vi "OverlayArrow.vi"(6 "Color":u32(colorbox)=16711680, 7 "GroupName":string, 8 "error in":errorcluster, 9 "Arrows":T1={"StartPoint"=TRUE, "StartArrowSize"=9.0, "EndPoint"=TRUE, "EndArrowSize"=9.0}, 10 "Line":T2, 11 "Image Reference In":T4) -> (0 "error out":errorcluster, 3 "Image Reference Out":T4)   [LabVIEW 2020, in "OpenLvVision_Overlays.lvlib"]
doc: "Overlays an Arrow into an image."
uses:
  OpenLvVision_Overlays.lvlib
  <vilib>/OpenLvVision/OpenLvVision_Image/Management/TypeDef/OLV Image.ctl
  TypeDefs/Line.ctl
  TypeDefs/PointI32.ctl
  TypeDefs/Arrows.ctl
  TypeDefs/DrawingMode.ctl
  <vilib>/OpenLvVision/OpenLvVision_Image/Management/OLV Management.lvlib
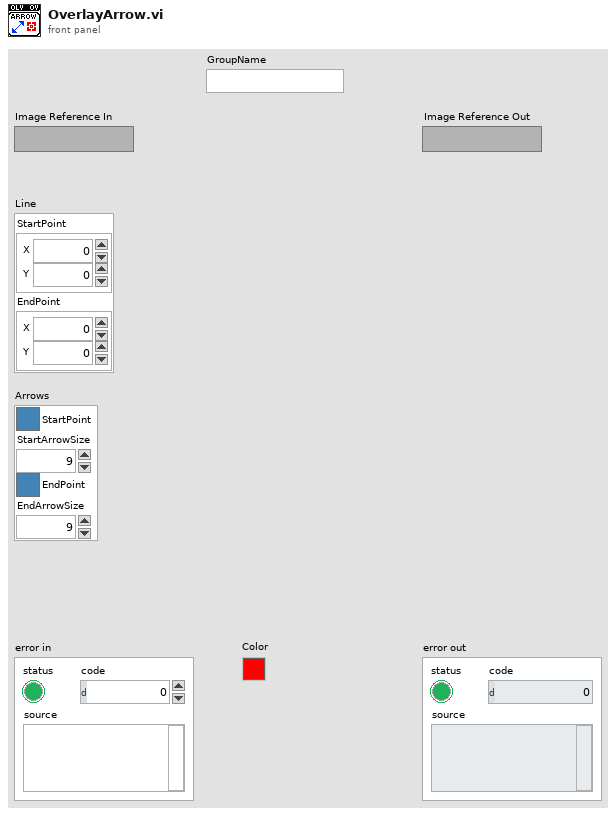
[diagram p1: front panel]
types:
  T1 = typedef "OpenLvVision_Overlays.lvlib/Arrows.ctl" = cluster{"StartPoint":bool, "StartArrowSize":dbl, "EndPoint":bool, "EndArrowSize":dbl}
  T2 = typedef "OpenLvVision_Overlays.lvlib/Line.ctl" = cluster{"StartPoint":T3, "EndPoint":T3}
  T3 = typedef "OpenLvVision_Overlays.lvlib/PointI32.ctl" = cluster{"X":i32, "Y":i32}
  T4 = typedef "OLV OpenLvVision_Image.lvlib/OLV Management.lvlib/OLV Image.ctl" = refnum<image>
  T5 = typedef "OpenLvVision_Overlays.lvlib/DrawingMode.ctl" = enum16{"Frame", "Fill"}
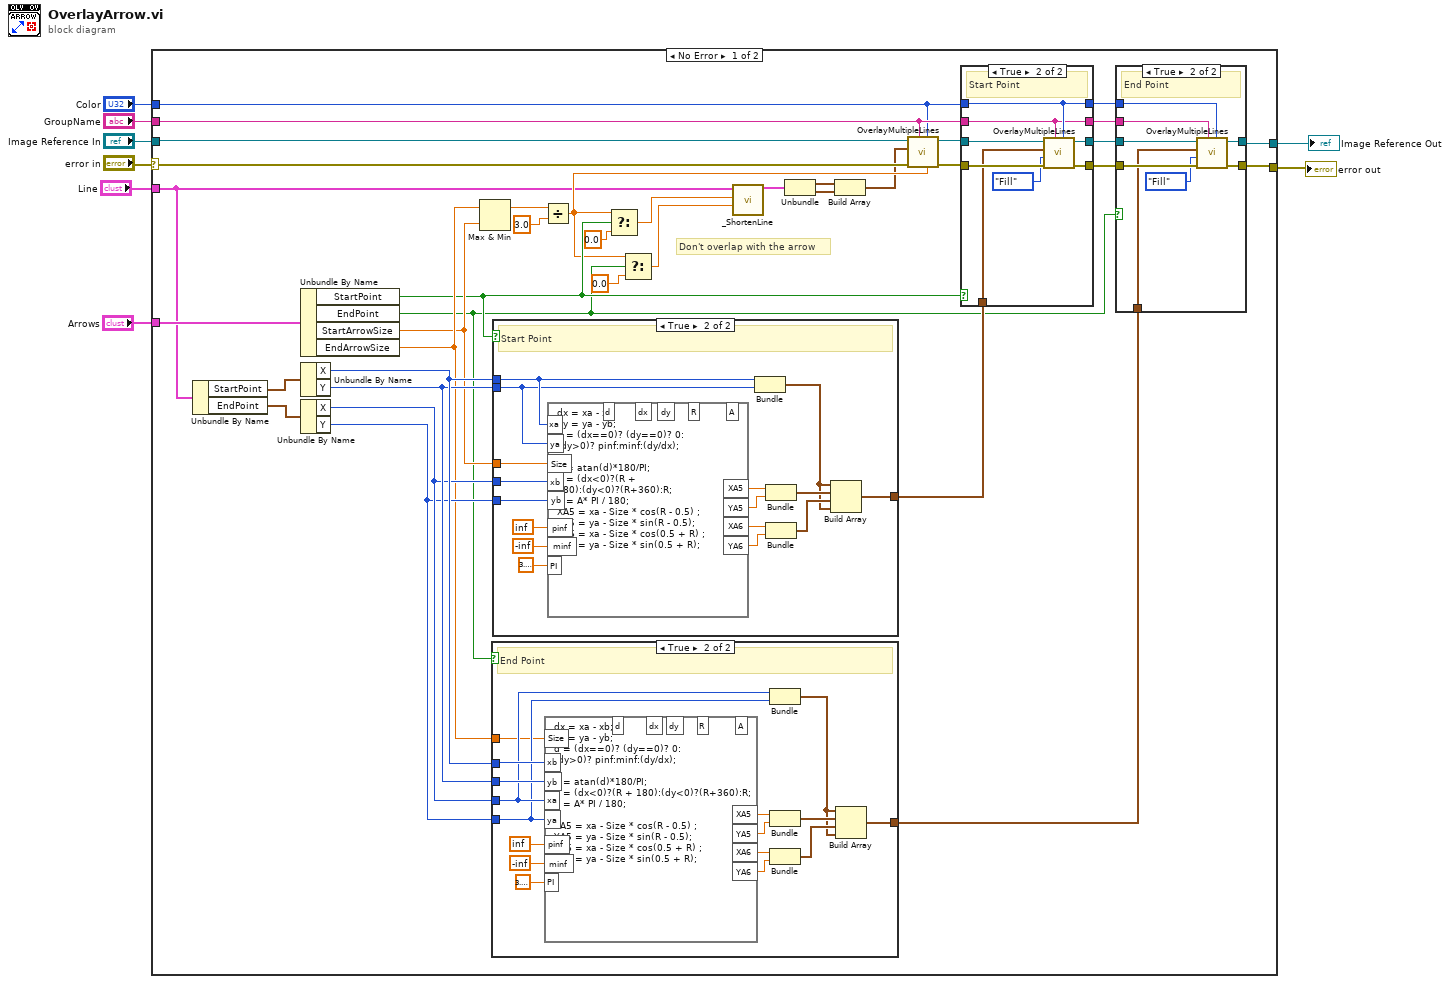
[diagram p0: block diagram]
diagram:
  n1 = case shown="No Error" "error in" {
    selector: "error in" -> [w32 w100]
    tunnel: [w36 w100] -> w7
    tunnel: "Image Reference In" -> [w31 w101]
    tunnel: [w35 w101] -> w6
    tunnel: "Arrows" -> [w45 _]
    tunnel: "Color" -> [w27 _]
    tunnel: "GroupName" -> [w28 _]
    tunnel: "Line" -> [w11 _]
    frame No Error {
      # "Don't overlap with the arrow"
      n2 = Unbundle By Name(w11) -> ("StartPoint"=w25:T3, "EndPoint"=w26:T3)
      n3 = Unbundle By Name(w45) -> ("StartPoint"=w19:bool, "EndPoint"=w18:bool, "StartArrowSize"=w21:dbl, "EndArrowSize"=w22:dbl)
      n4 = Unbundle By Name(w25) -> ("X"=w44:i32, "Y"=w43:i32)
      n5 = Unbundle By Name(w26) -> ("X"=w42:i32, "Y"=w41:i32)
      n6 = Max & Min(x=w22, y=w21) -> (max(x,y)=w13:dbl)  [unwired: 1 out]
      n7 = case shown="True" w18 {
        tunnel: w44 -> [_ w70]
        tunnel: w43 -> [_ w69]
        tunnel: w42 -> [_ w68]
        tunnel: w41 -> [_ w67]
        tunnel: [_ w59] -> w33
        tunnel: w22 -> [_ w58]
        frame False {
        }
        frame True {
          # "End Point"
          n8 = formula code="dx = xa - xb;\ndy = ya - yb;\nd = (dx==0)? (dy==0)? 0:\n(dy>0)? pinf:minf:(dy/dx);\n\nR = atan(d)*180/PI;\nA = (dx<0)?(R + 180):(dy<0)?(R+360):R;\nR = A* PI / 180;\n\nXA5 = xa - Size * cos(R - 0.5) ;\nYA5 = ya - Size * sin(R - 0.5);\nXA6 = xa - Size * cos(0.5 + R) ;\nYA6 = ya - Size * sin(0.5 + R);"("xb"=w70, "yb"=w69, "xa"=w68, "ya"=w67, "pinf"=inf, "minf"=-inf, "PI"=3.141592653589793, "Size"=w58) -> ("XA5"=w66:dbl, "YA5"=w65:dbl, "XA6"=w64:dbl, "YA6"=w63:dbl)  [unwired: 5 out]
          n9 = Bundle("X"=w68, "Y"=w67) -> (w60:cluster{"X":i32, "Y":i32})  [unwired: 1 out]
          n10 = Bundle("XA5"=w66, "YA5"=w65) -> (w62:cluster{"XA5":dbl, "YA5":dbl})  [unwired: 1 out]
          n11 = Bundle("XA6"=w64, "YA6"=w63) -> (w61:cluster{"XA6":dbl, "YA6":dbl})  [unwired: 1 out]
          n12 = Build Array(w60, w62, w61, w60) -> (w59:cluster{"XA6":dbl, "YA6":dbl}[])
        }
      }
      n13 = case shown="True" w19 {
        tunnel: w44 -> [_ w78]
        tunnel: w43 -> [_ w77]
        tunnel: w42 -> [_ w79]
        tunnel: w41 -> [_ w76]
        tunnel: [_ w75] -> w34
        tunnel: w21 -> [_ w74]
        frame False {
        }
        frame True {
          # "Start Point"
          n14 = formula code="dx = xa - xb;\ndy = ya - yb;\nd = (dx==0)? (dy==0)? 0: \n(dy>0)? pinf:minf:(dy/dx);\n\nR = atan(d)*180/PI;\nA = (dx<0)?(R + 180):(dy<0)?(R+360):R;\nR = A* PI / 180;\nXA5 = xa - Size * cos(R - 0.5) ;\nYA5 = ya - Size * sin(R - 0.5);\nXA6 = xa - Size * cos(0.5 + R) ;\nYA6 = ya - Size * sin(0.5 + R);"("xa"=w78, "ya"=w77, "xb"=w79, "yb"=w76, "pinf"=inf, "minf"=-inf, "PI"=3.141592653589793, "Size"=w74) -> ("XA5"=w86:dbl, "YA5"=w85:dbl, "XA6"=w84:dbl, "YA6"=w83:dbl)  [unwired: 5 out]
          n15 = Bundle("X"=w78, "Y"=w77) -> (w80:cluster{"X":i32, "Y":i32})  [unwired: 1 out]
          n16 = Bundle("XA5"=w86, "YA5"=w85) -> (w82:cluster{"XA5":dbl, "YA5":dbl})  [unwired: 1 out]
          n17 = Bundle("XA6"=w84, "YA6"=w83) -> (w81:cluster{"XA6":dbl, "YA6":dbl})  [unwired: 1 out]
          n18 = Build Array(w80, w82, w81, w80) -> (w75:cluster{"XA6":dbl, "YA6":dbl}[])
        }
      }
      n19 = Divide(x=w13, y=3.0) -> (x/y=w15:dbl)
      n20 = Select(t=w15, s=w19, f=0.0) -> (s? t:f=w10:dbl)
      n21 = Select(t=w15, s=w18, f=0.0) -> (s? t:f=w9:dbl)
      n22 = call "_ShortenLine.vi"("ShortEnd"=w9, "ShortStart"=w10, "Line"=w11) -> ("Line"=w12:T2)  [unwired: 8 in]
      n23 = Unbundle(w12) -> ("StartPoint"=w24:T3, "EndPoint"=w23:T3)
      n24 = Build Array(w24, w23) -> (w14:T3[])
      n25 = call "OverlayMultipleLines.vi"("Width"=w15, "Color"=w27, "GroupName"=w28, "error in"=w32, "Points"=w14, "Image Reference In"=w31) -> ("error out"=w29:errorcluster, "Image Reference Out"=w30:T4)  [unwired: 4 in]
      n26 = case shown="True" w19 {
        tunnel: w30 -> [w48 w57]
        tunnel: w29 -> [w46 w56]
        tunnel: [w48 w55] -> w38
        tunnel: [w46 w54] -> w37
        tunnel: w28 -> [w47 w52]
        tunnel: w27 -> [w49 w53]
        tunnel: [w49 w53] -> w40
        tunnel: [w47 w52] -> w39
        tunnel: w34 -> [_ w51]
        frame False {
        }
        frame True {
          # "Start Point"
          n27 = call "OverlayMultipleLines.vi"("Color"=w53, "GroupName"=w52, "error in"=w56, "Drawing Mode (Frame)"=DrawingMode."Fill", "Points"=w51, "Image Reference In"=w57) -> ("error out"=w54:errorcluster, "Image Reference Out"=w55:T4)  [unwired: 4 in]
        }
      }
      n28 = case shown="True" w18 {
        tunnel: w38 -> [w91 w99]
        tunnel: w37 -> [w90 w98]
        tunnel: [w91 w97] -> w35
        tunnel: [w90 w96] -> w36
        tunnel: w39 -> [_ w94]
        tunnel: w40 -> [_ w95]
        tunnel: w33 -> [_ w93]
        frame False {
        }
        frame True {
          # "End Point"
          n29 = call "OverlayMultipleLines.vi"("Color"=w95, "GroupName"=w94, "error in"=w98, "Drawing Mode (Frame)"=DrawingMode."Fill", "Points"=w93, "Image Reference In"=w99) -> ("error out"=w96:errorcluster, "Image Reference Out"=w97:T4)  [unwired: 4 in]
        }
      }
    }
    frame Error {
    }
  }
  "error out" <- w7
  "Image Reference Out" <- w6
